vi "PicoScopeospaGetNoOfProcessedCaptures.vi"(8 "error in (no error)":errorcluster, 11 "handle in":i16=16384) -> (0 "error out":errorcluster, 3 "handle out":i16, 6 "nCaptures":u64)   [LabVIEW 2010]
doc: "This function returns the number of captures collected in one run of rapid block mode. You can call this function during device capture, after collection has completed or after interrupting waveform collection by calling psospaStop().\n\nThe returned value (nCaptures) can then be used to iterate through the number of segments using psospaGetValues(), or in a single call to psospaGetValuesBulk() where it is used to calculate the toSegmentIndex parameter."
uses:
  psospa.dll
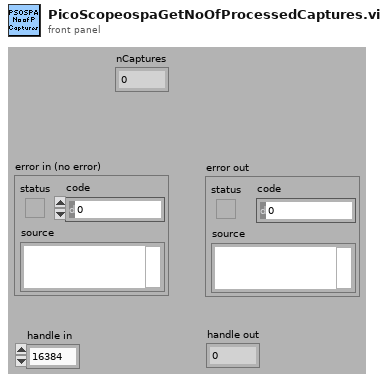
[diagram p1: front panel]
types:
  T1 = cluster{"status":bool, "code":u32, "source":string}
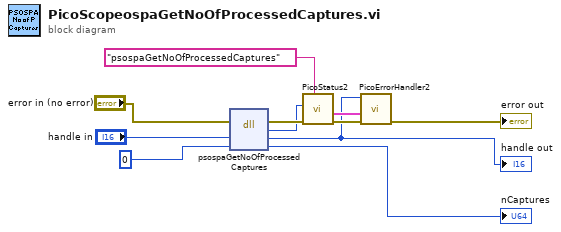
[diagram p0: block diagram]
diagram:
  n1 = dll-call lib="psospa.dll" fn="psospaGetNoOfProcessedCaptures"(error in="error in (no error)", "handle"="handle in", "nCaptures"=u64 0) -> (error out=w7:errorcluster, "PICO_STATUS"=w5:u32, "handle"=w4:i16, "nCaptures"=→"nCaptures":u64)  [unwired: 2 in, 1 out]
  "handle out" <- w4
  n2 = call "PicoStatus2.vi"("PICO source"="psospaGetNoOfProcessedCaptures" ("source"), "Error in"=w7, "PICO STATUS"=w5) -> ("error out"=w8:errorcluster, "PICO_STATUS out"=w9:T1)  [unwired: 5 in]
  n3 = call "PicoErrorHandler2.vi"("error in (no error)"=w8, "PICO_STATUS in"=w9, "handle In"=w4) -> ("error out"=→"error out":errorcluster)  [unwired: 8 in]
